vi "Search_register_path.vi"(8 "error in (no error)":errorcluster caption="错误输入（无错误）", 11 "Path_management 输入":refnum<class "Path_management.lvclass">) -> (0 "error out":errorcluster caption="错误输出", 2 "路径数组":path[](array[path]), 3 "Path_management 输出":refnum<class "Path_management.lvclass">)   [LabVIEW 2025, in "Path_management.lvclass"]
uses:
  Path_management.lvclass
  Register_path.ctl
  Path_management.lvclass/Path_management.ctl
panel:
  in  "组合框":T1
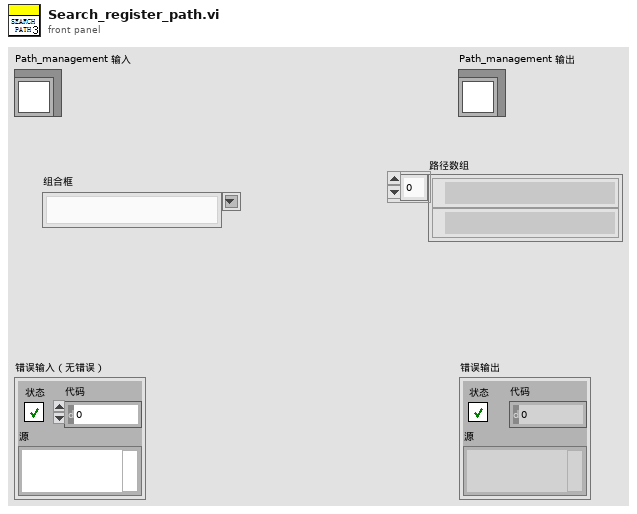
[diagram p1: front panel]
types:
  T1 = typedef "Path_management.lvclass/Register_path.ctl" = string
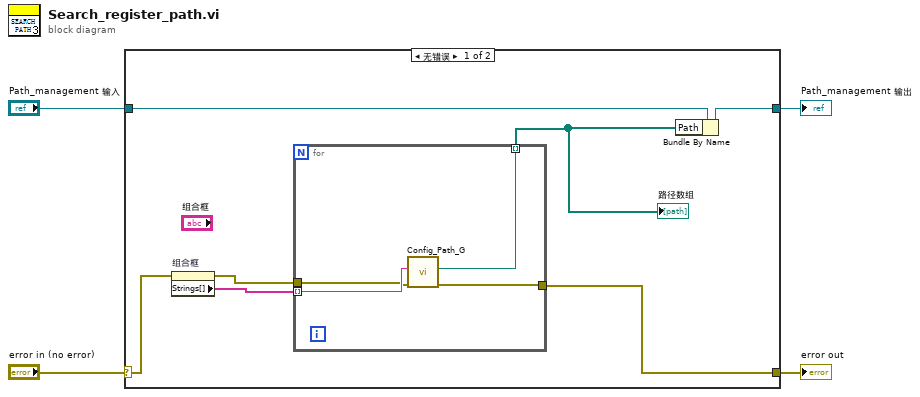
[diagram p0: block diagram]
diagram:
  n1 = case shown="无错误" "error in (no error)" {
    selector: "error in (no error)" -> [w10 w17]
    tunnel: [w5 w17] -> w3
    tunnel: [w8 w16] -> w1
    tunnel: "Path_management 输入" -> [w11 w16]
    frame No Error {
      n2 = property on="组合框" class="CmbBox (严格)"(error in=w10) -> (error out=w6:errorcluster, "Strings[]"=w9:string[])  [unwired: 1 in, 1 out]
      n3 = for {
        tunnel: w9 -> [w15] mode=indexing
        tunnel: [w14] -> w7 mode=indexing
        tunnel: w6 -> [w13]
        tunnel: [w12] -> w5
        n4 = call "Config_Path_G.vi"("error in (no error)"=w13, "pattern"=w15) -> ("error out"=w12:errorcluster, "路径"=w14:path)  [unwired: 8 in]
      }
      "路径数组" <- w7
      n5 = Bundle By Name(cluster=w11, "Path"=w7) -> (w8:refnum<class "Path_management.lvclass">)
    }
    frame Error {
    }
  }
  "error out" <- w3
  "Path_management 输出" <- w1
